vi "ReversedEngineering GetCompleteDependencyInfo.vi"(1 "path":path[](array[path]), 2 "SearchElements":T2[](array[typedef]), 4 "IgnoreClasses":path[](array[path]), 5 "error in (no error)":errorcluster, 6 "Only Create this class and its dependencis":bool, 7 "SyncOption":T1, 8 "Only analyse this class methods and attributes(False)":bool, 10 "CreateApplicationNode":bool) -> (15 "classInfos":T7[](array[typedef]), 16 "TypeDefs":T3[](array[typedef]), 17 "Cancelled":bool, 19 "error out":errorcluster)   [LabVIEW 2020]
doc: "Gets current diagram values"
uses:
  <resource>/Framework/Providers/Open_GDS/UML/ReversedEngineering/ReversedEngineering ClassInfoType.ctl
  <resource>/Framework/Providers/Open_GDS/ClassProviders/Common/CommonVIs/CommonVIs_VisibilityType.ctl
  <resource>/Framework/Providers/Open_GDS/ClassProviders/Common/CommonVIs/CommonVIs_AttributeInfoType.ctl
  <resource>/Framework/Providers/Open_GDS/ClassProviders/Common/CommonVIs/CommonVIs_AttributeDataType.ctl
  <resource>/Framework/Providers/Open_GDS/UML/ReversedEngineering/ReversedEngineering_ClassDependencyDetailsType.ctl
  <resource>/Framework/Providers/Open_GDS/ClassProviders/Common/ScriptingFunctions/SubVIs/Scripting_ViDependencyType.ctl
  <resource>/Framework/Providers/Open_GDS/ClassProviders/Common/CommonVIs/CommonVIs_TypeDefType.ctl
  <resource>/Framework/Providers/Open_GDS/UML/ReversedEngineering/ReversedEngineering RecursiveSearchElements.ctl
  <resource>/Framework/Providers/Open_GDS/UML/UMLEditor/UMLEditor_SyncOptions.ctl
  <resource>/Framework/Providers/Open_GDS/UML/UMLEditor/UMLEditor BusyDialogAction.ctl
  <resource>/Framework/Providers/Open_GDS/UML/UmlEditor_class/UmlEditor.lvclass
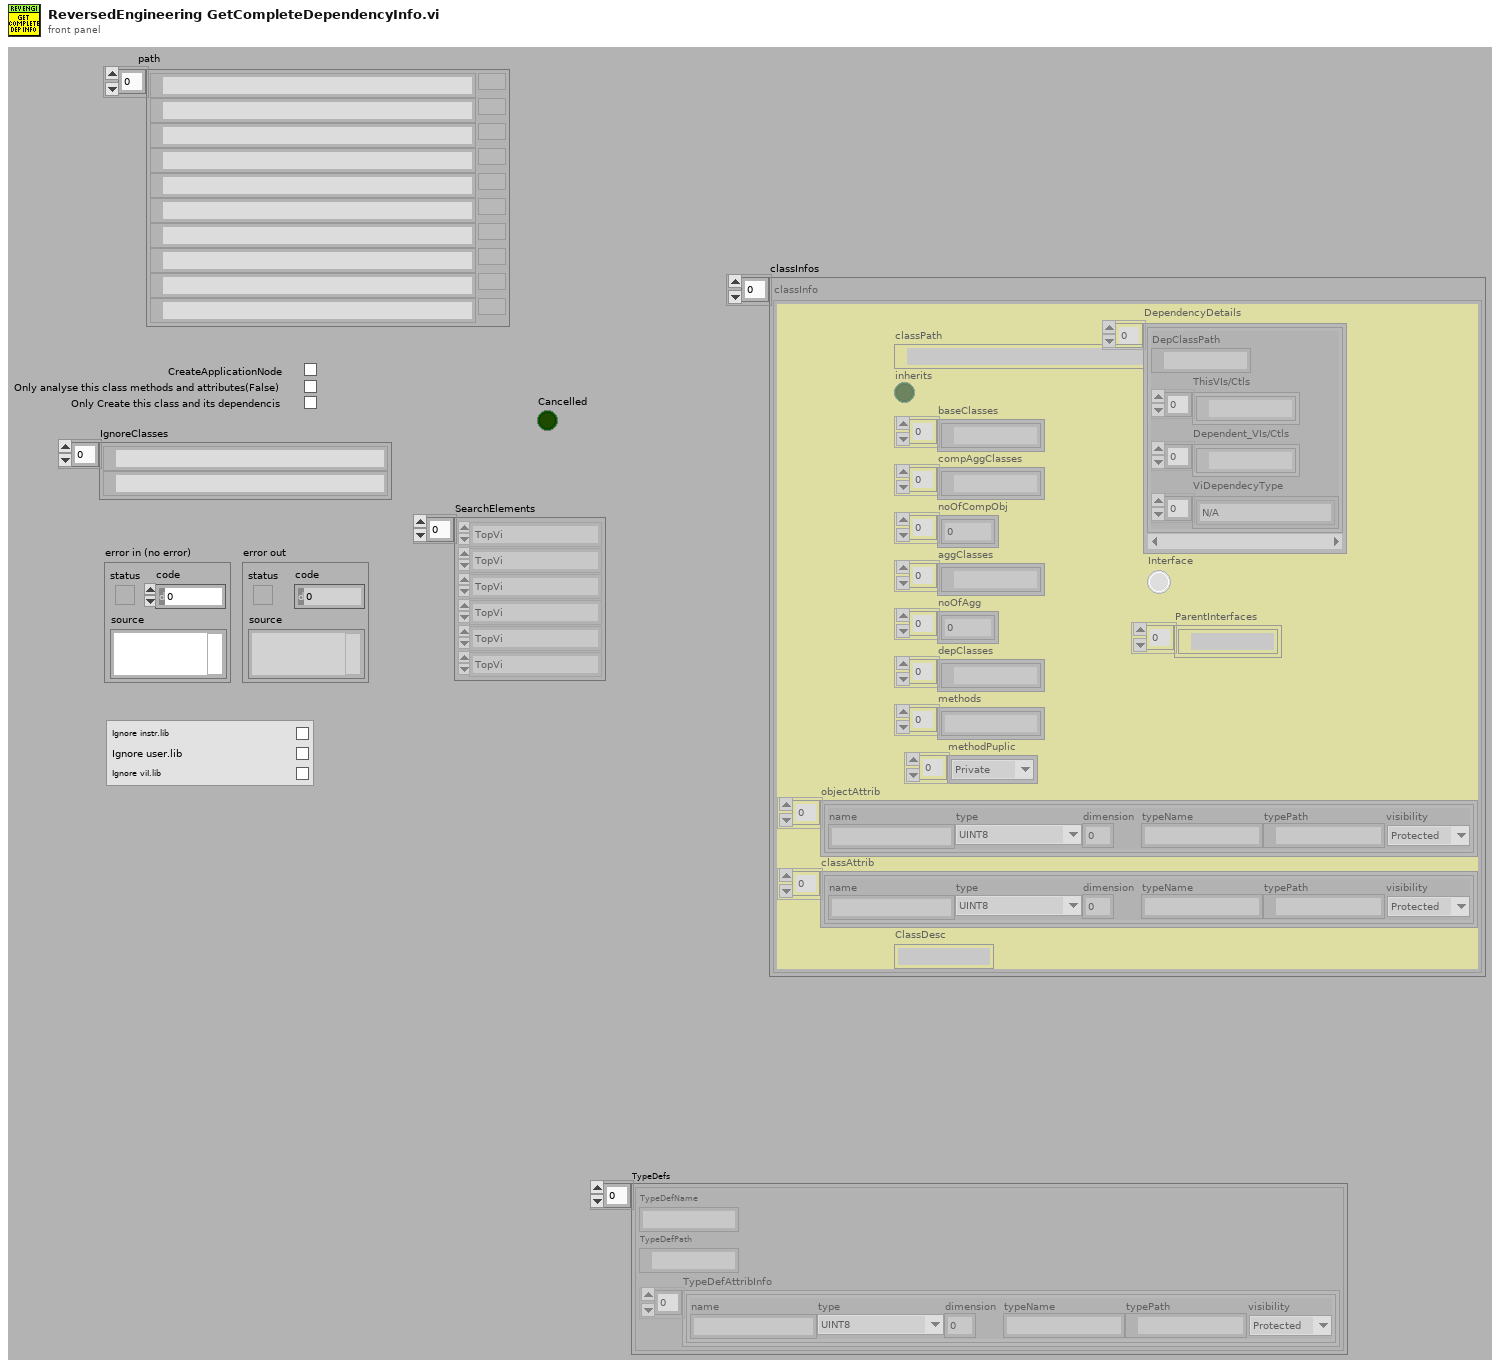
[diagram p1: front panel]
types:
  T1 = typedef "UMLEditor_SyncOptions.ctl" = cluster{"IgnoreInstrLib":bool, "IgnoreUserLib":bool, "IgnoreViLib":bool}
  T2 = typedef "ReversedEngineering RecursiveSearchElements.ctl" = enum16{"TopVi", "Class", "Dir", "Dir(rec.)"}
  T3 = typedef "CommonVIs_TypeDefType.ctl" = cluster{"TypeDefName":string, "TypeDefPath":path, "TypeDefAttribInfo":T4[]}
  T4 = typedef "CommonVIs_AttributeInfoType.ctl" = cluster{"name":string, "type":T5, "dimension":i32, "typeName":string, "typePath":path, "visibility":T6}
  T5 = typedef "CommonVIs_AttributeDataType.ctl" = enum16{"UINT8", "INT8", "UINT16", "INT16", "UINT32", "INT32", "UINT64", "INT64", "SGL", "DBL", "EXT", "CSG", "CDB", "CXT", "TimeStamp", "STRING", "PATH", "BOOL", "ENUM", "RefNum", "VIRefNum", "LabVIEW Class", "Cluster", "Variant", "TypeDef", "Waveform", "LabVIEW Object", "Other", "void", "Set", "Map"}
  T6 = typedef "CommonVIs_VisibilityType.ctl" = enum16{"Public", "Private", "Protected"}
  T7 = typedef "ReversedEngineering ClassInfoType.ctl" = cluster{"classPath":path, "inherits":bool, "baseClasses":path[], "compAggClasses":path[], "noOfCompObj":i32[], "aggClasses":path[], "noOfAgg":i32[], "depClasses":path[], "methods":string[], "methodPuplic":T6[], "objectAttrib":T4[], "classAttrib":T4[], "ClassDesc":string, "DependencyDetails":T8[], "Interface":bool, "ParentInterfaces":path[]}
  T8 = typedef "ReversedEngineering_ClassDependencyDetailsType.ctl" = cluster{"DepClassPath":path, "ThisVIs/Ctls":path[], "Dependent_VIs/Ctls":path[], "ViDependecyType":T9[]}
  T9 = typedef "Scripting_ViDependencyType.ctl" = enum16{"N/A", "Launches"}
  T10 = cluster{"dependencyClassPath":path[], "topVIPath":path, "classInfos":T7[], "calleesVIs":path[], "VIRef":refnum<vi>[], "TypeDefs":T3[], "TopVIPath":path, "SearchOnlyClasses":bool, "SearchDirs":path[], "SearchOnlyTopVIs":bool, "lvclasses":path[]}
  T11 = enum16{"Get Library Info", "Create Library Info", "Clear Library Info"}
  T12 = typedef "UMLEditor BusyDialogAction.ctl" = enum16{"Initialize", "Open(VIs)", "Open(i)", "Send_I-Value", "SendStatusMessage", "GetBusyDialogStatus", "Close", "Quit"}
  T13 = typedef "Librarian File Info Out.ctl" = cluster{"creation date":u32, "last mod date":u32, "type":string, "creator":string, "LV version":i32, "size":i32, "top level":bool}
  T14 = typedef "Scripting_VIClassDependency.ctl" = cluster{"VIPath":path, "Class":string, "ClassPath":path, "ViDependencyType":T9}
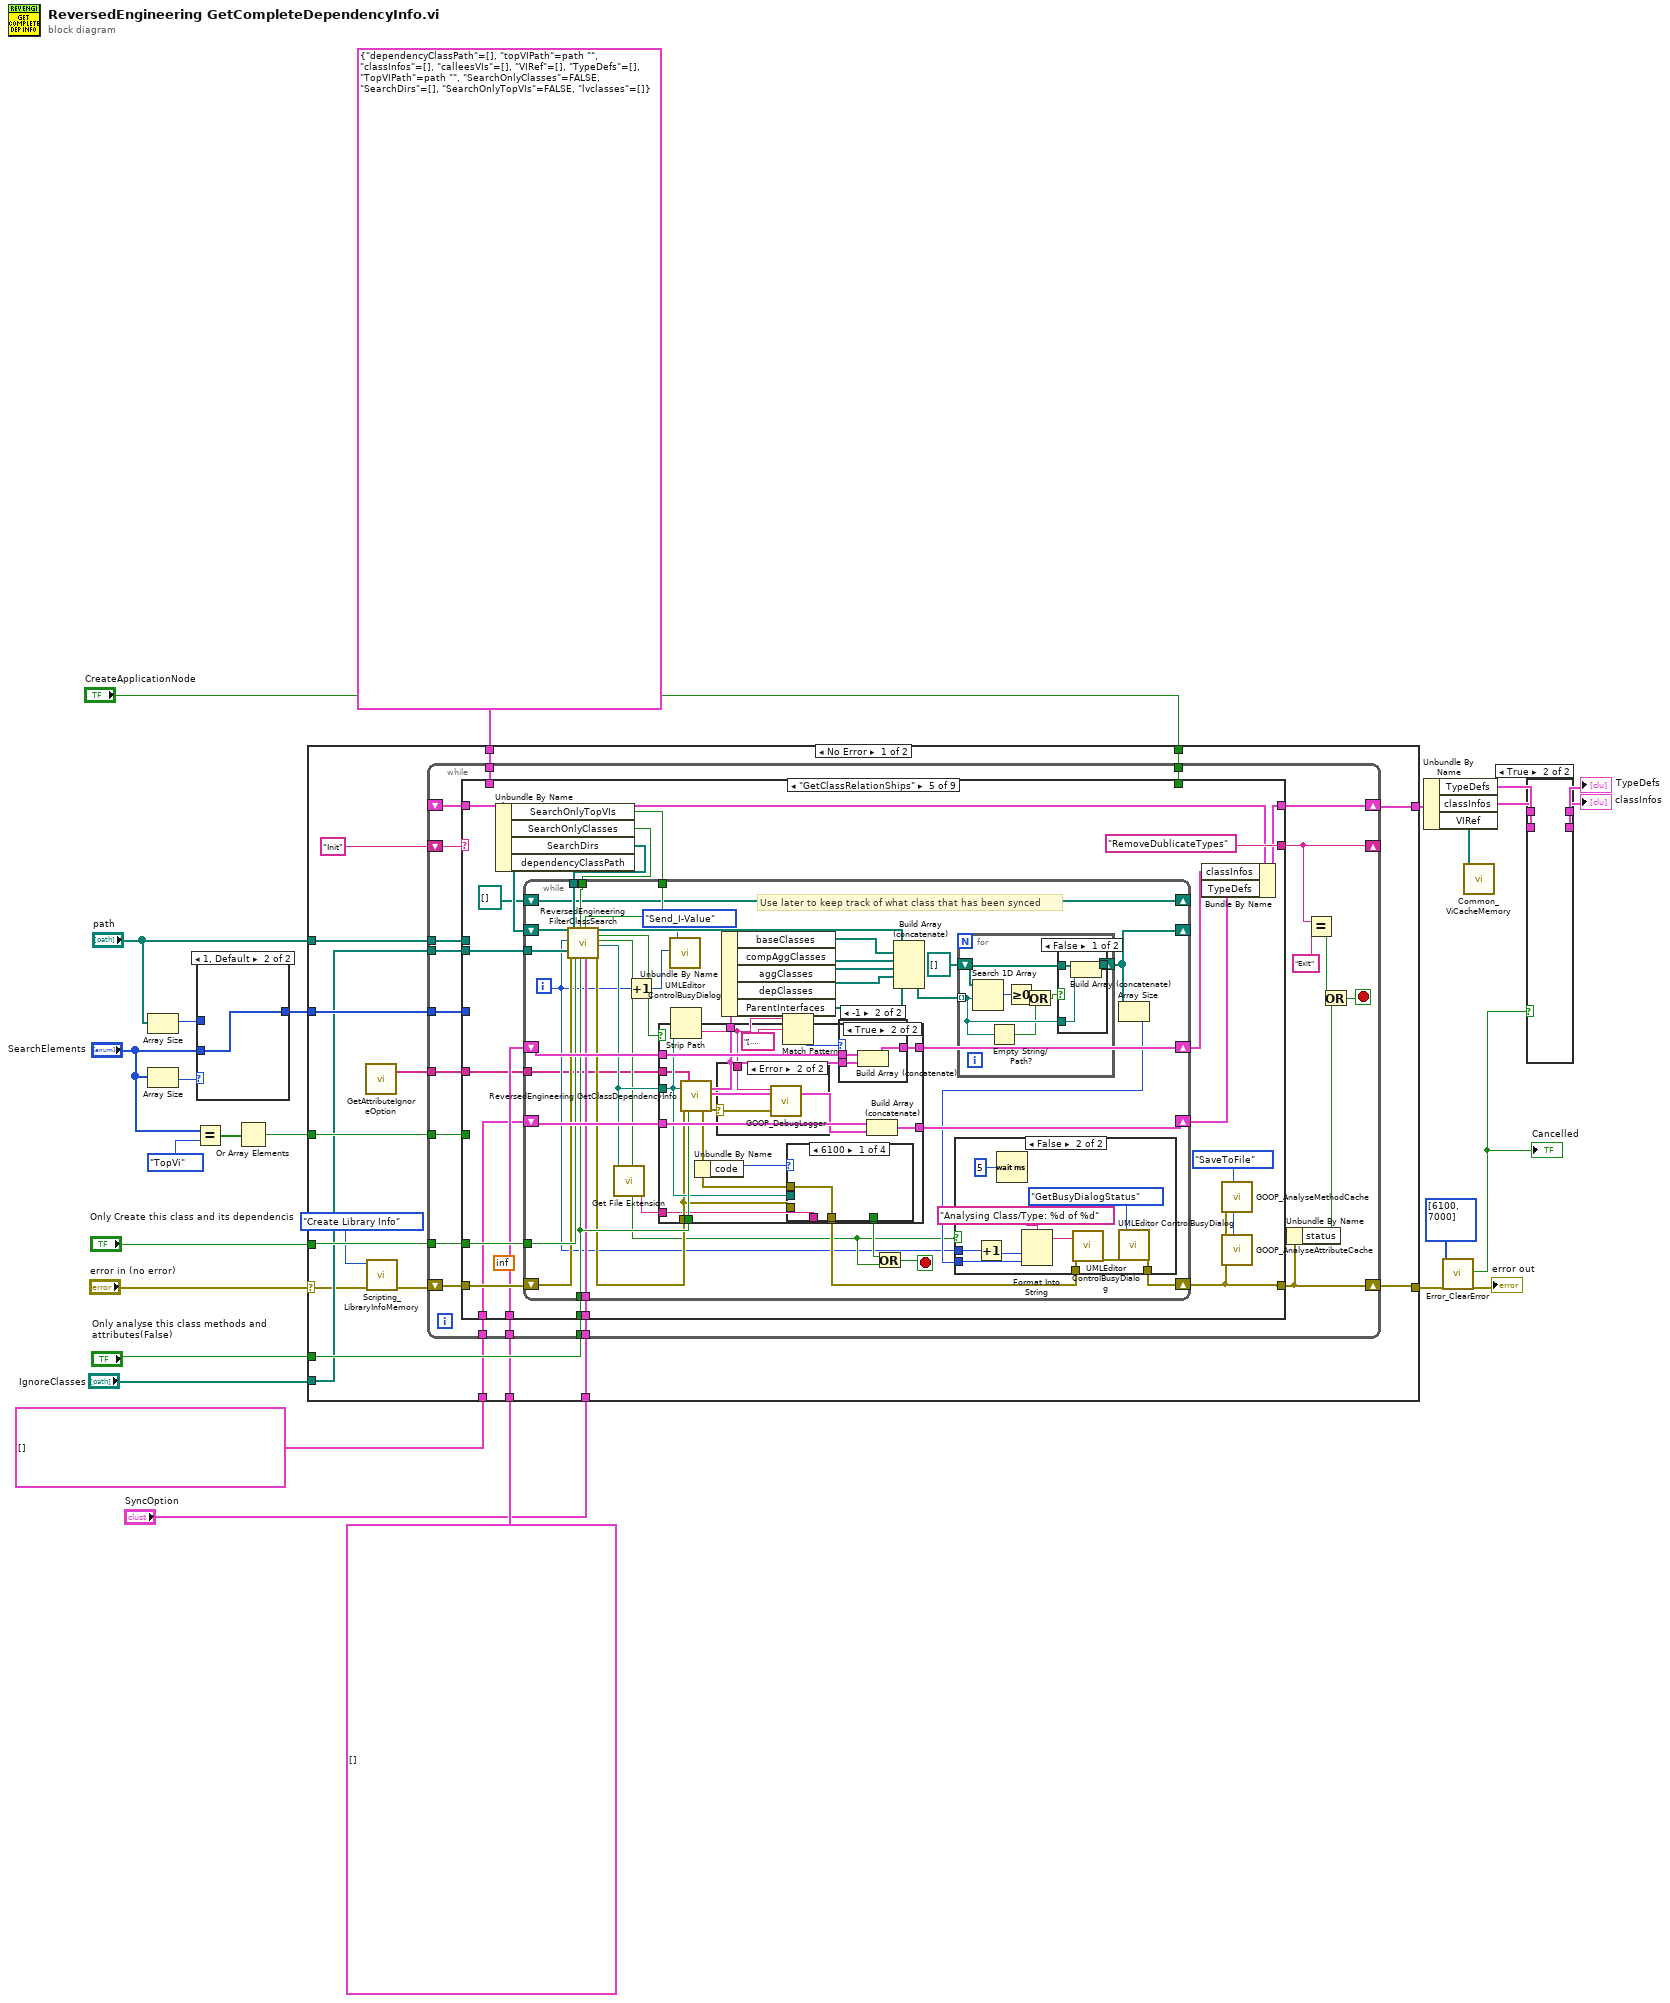
[diagram p0: block diagram]
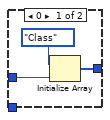
[diagram p3: hidden frame]
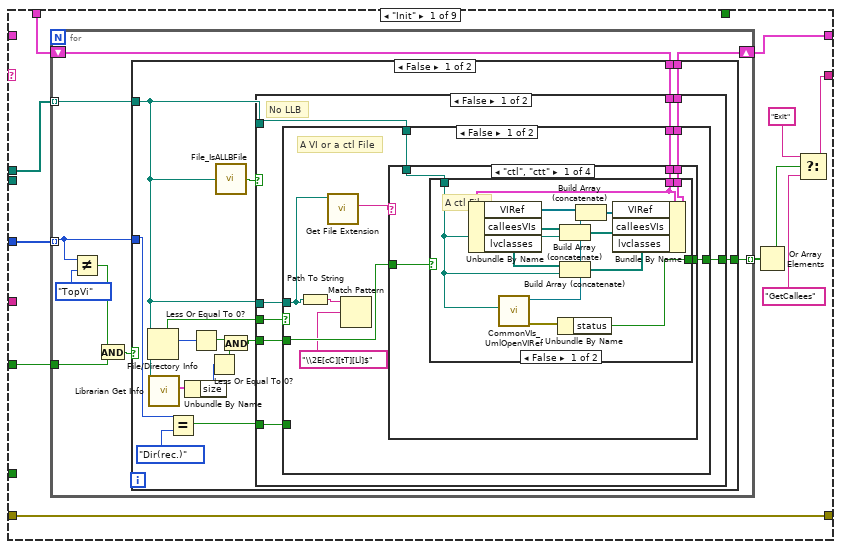
[diagram p4: hidden frame]
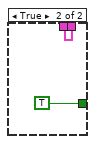
[diagram p5: hidden frame]
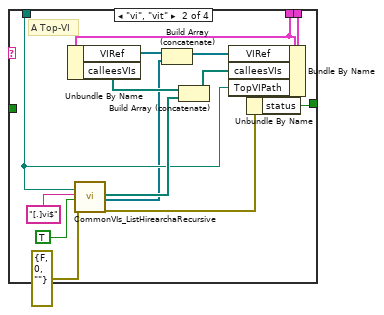
[diagram p6: hidden frame]
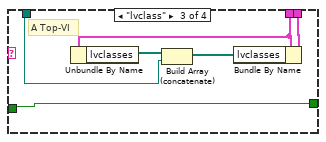
[diagram p7: hidden frame]
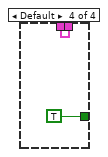
[diagram p8: hidden frame]
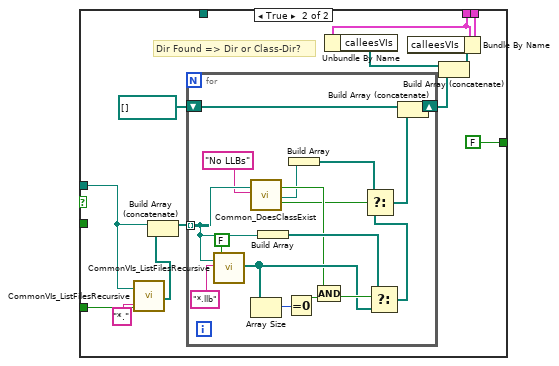
[diagram p9: hidden frame]
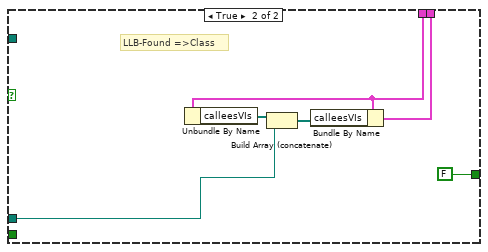
[diagram p10: hidden frame]
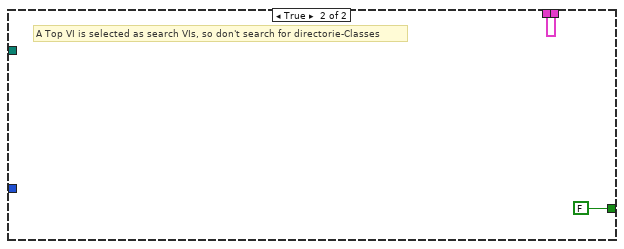
[diagram p11: hidden frame]
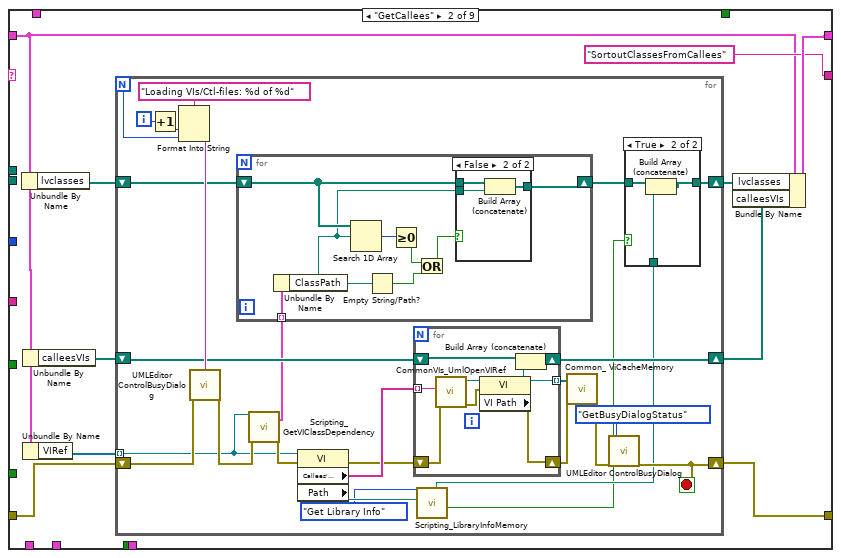
[diagram p12: hidden frame]
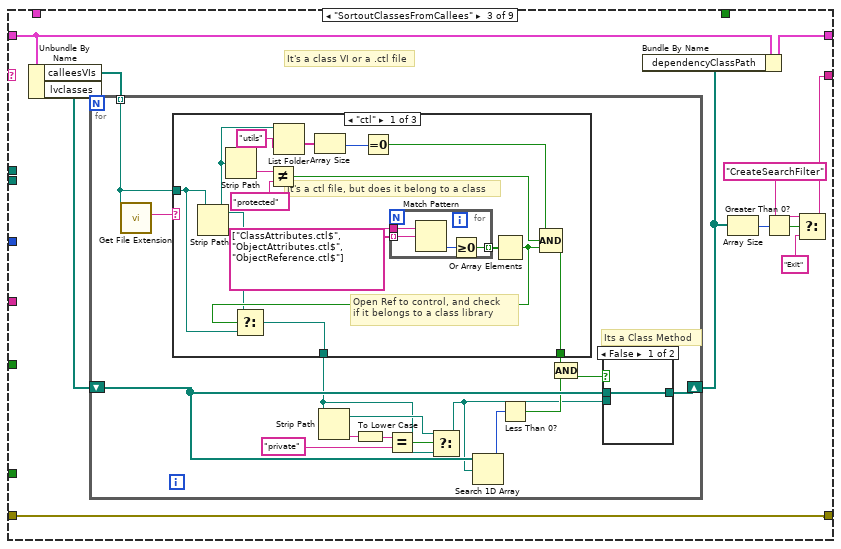
[diagram p15: hidden frame]
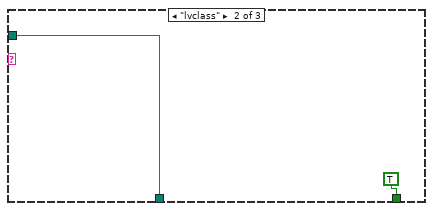
[diagram p16: hidden frame]
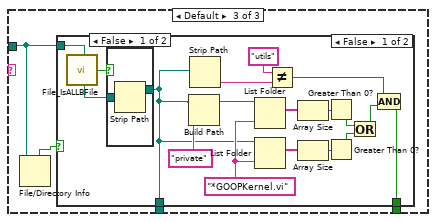
[diagram p17: hidden frame]
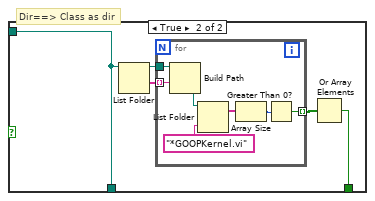
[diagram p19: hidden frame]
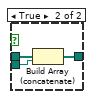
[diagram p20: hidden frame]
diagram:
  n1 = Array Size(array="path") -> (size(s)=w19:i32)
  n2 = Array Size(array="SearchElements") -> (size(s)=w21:i32)
  n3 = Equal?(x="SearchElements", y=ReversedEngineering_RecursiveSearchElements."TopVi" ("Enum")) -> (x = y?=w9:bool[])
  n4 = case shown="1, Default" w21 {
    tunnel: w19 -> [w29 _]
    tunnel: [w28 w31] -> w18
    tunnel: "SearchElements" -> [_ w31]
    frame 0 {
      n5 = Initialize Array(ReversedEngineering_RecursiveSearchElements."Class" ("Enum"), w29) -> (w28:T2[])
    }
    frame 1, Default {
    }
  }
  n6 = Or Array Elements(Boolean array=w9) -> (logical OR=w7:bool)
  n7 = case shown="No Error" "error in (no error)" {
    selector: "error in (no error)" -> [w35 w642]
    tunnel: [w48 w642] -> w17
    tunnel: "path" -> [w47 _]
    tunnel: [w46 _] -> w26
    tunnel: "Only Create this class and its dependencis" -> [w45 _]
    tunnel: "Only analyse this class methods and attributes(False)" -> [w42 _]
    tunnel: "CreateApplicationNode" -> [w44 _]
    tunnel: w18 -> [w43 _]
    tunnel: w7 -> [w41 _]
    tunnel: T10 {"dependencyClassPath"=[], "topVIPath"=path "", "classInfos"=[], "calleesVIs"=[], "VIRef"=[], "TypeDefs"=[], "TopVIPath"=path "", "SearchOnlyClasses"=FALSE, "SearchDirs"=[], "SearchOnlyTopVIs"=FALSE, "lvclasses"=[]} ("Cluster") -> [w40 _]
    tunnel: T7[] [] -> [w39 _]
    tunnel: T3[] [] -> [w38 _]
    tunnel: "IgnoreClasses" -> [w37 _]
    tunnel: "SyncOption" -> [w36 _]
    frame No Error {
      n8 = call <resource>:"GetAttributeIgnoreOption.vi"() -> ("Attr"=w32:string[])  [unwired: 1 in, 18 out]
      n9 = call <resource>:"Scripting_LibraryInfoMemory.vi"("error in (no error)"=w35, "Action"=T11."Create Library Info") -> ("error out"=w34:errorcluster)  [unwired: 5 in, 4 out]
      n10 = while {
        shift-right: [w68] -> _
        shift-left: "Init" -> [w71]
        shift-right: [w69] -> w48
        shift-left: w34 -> [w70]
        shift-right: [w62] -> w46
        shift-left: _ -> [w63]
        tunnel: w47 -> [w61]
        tunnel: w45 -> [w60]
        tunnel: w44 -> [w59]
        tunnel: w43 -> [w58]
        tunnel: w42 -> [w57]
        tunnel: w41 -> [w56]
        tunnel: w40 -> [w55]
        tunnel: w39 -> [w54]
        tunnel: w38 -> [w53]
        tunnel: w37 -> [w52]
        tunnel: w36 -> [w51]
        tunnel: w32 -> [w50]
        stop <- w64 stop-if-true
        n11 = case shown="\"GetClassRelationShips\"" w71 {
          tunnel: w70 -> [w82 w207 w271 w353 w419 w528 w559 w631 w639]
          tunnel: [w82 w208 w271 w350 w405 w528 w559 w631 w639] -> w69
          tunnel: [w81 "SortoutClassesFromCallees" ("y") w266 "GetClassRelationShips" ("y") "RemoveDublicateTypes" ("y") "RemoveClassDependenciesDueToInheritance" ("y") w555 "Exit" ("y") "Exit" ("y")] -> w68
          tunnel: w63 -> [_ w204 w270 w365 w420 w531 w561 w630 w641]
          tunnel: [w75 w210 w272 w364 w421 w529 w560 w629 w641] -> w62
          tunnel: w61 -> [w80 _ _ w360 _ _ _ _ _]
          tunnel: w60 -> [_ _ _ _ w416 _ _ _ _]
          tunnel: w59 -> [_ _ _ _ _ _ w553 _ _]
          tunnel: w58 -> [w74 _ _ w355 _ _ _ _ _]
          tunnel: w57 -> [_ _ _ _ w414 _ _ _ _]
          tunnel: w56 -> [w73 _ _ _ _ _ _ _ _]
          tunnel: w55 -> [w72 _ _ _ _ _ _ _ _]
          tunnel: w54 -> [_ _ _ _ w410 _ _ _ _]
          tunnel: w53 -> [_ _ _ _ w409 _ _ _ _]
          tunnel: w52 -> [_ _ _ _ w407 _ _ _ _]
          tunnel: w51 -> [_ _ _ _ w406 _ _ _ _]
          tunnel: w50 -> [_ _ _ _ w403 _ _ _ _]
          frame "Init" {
            n12 = for {
              tunnel: w80 -> [w88] mode=indexing
              shift-right: [w90] -> w75
              shift-left: w72 -> [w91]
              tunnel: [w89] -> w79 mode=indexing
              tunnel: w74 -> [w87] mode=indexing
              tunnel: w73 -> [w83]
              n13 = Not Equal?(x=w87, y=ReversedEngineering_RecursiveSearchElements."TopVi") -> (x != y?=w85:bool)
              n14 = And(x=w85, y=w83) -> (x .and. y?=w84:bool)
              n15 = case shown="False" w84 {
                tunnel: w91 -> [w106 w200]
                tunnel: [w105 w200] -> w90
                tunnel: [w104 FALSE ("status")] -> w89
                tunnel: w88 -> [w96 _]
                tunnel: w87 -> [w99 _]
                frame False {
                  n16 = File/Directory Info(path=w96) -> (directory=w102:bool, size=w98:i64)  [unwired: 1 in, 5 out]
                  n17 = call <vilib>:"Librarian Get Info.vi"("path"=w96) -> ("file information"=w95:T13)  [unwired: 1 in, 9 out]
                  n18 = Equal?(x=w99, y=ReversedEngineering_RecursiveSearchElements."Dir(rec.)") -> (x = y?=w100:bool)
                  n19 = Unbundle By Name(w95) -> ("size"=w94:i32)
                  n20 = Less Or Equal To 0?(x=w98) -> (x <= 0?=w97:bool)
                  n21 = Less Or Equal To 0?(x=w94) -> (x <= 0?=w93:bool)
                  n22 = call <resource>:"File_IsALLBFile.vi"("path"=w96) -> ("path to VI library?"=w103:bool)
                  n23 = And(x=w97, y=w93) -> (x .and. y?=w92:bool)
                  n24 = case shown="False" w103 {
                    tunnel: w92 -> [w114 _]
                    tunnel: w96 -> [w113 _]
                    tunnel: w106 -> [w112 w196]
                    tunnel: [w111 w197] -> w105
                    tunnel: [w110 FALSE ("status")] -> w104
                    tunnel: w96 -> [w108 w195]
                    tunnel: w102 -> [w109 _]
                    tunnel: w100 -> [w107 _]
                    frame False {
                      # "No LLB"
                      n25 = case shown="False" w109 {
                        tunnel: w114 -> [w123 _]
                        tunnel: w113 -> [w122 _]
                        tunnel: w112 -> [w121 w174]
                        tunnel: [w120 w173] -> w111
                        tunnel: [w119 FALSE] -> w110
                        tunnel: w108 -> [w116 w169]
                        tunnel: w107 -> [_ w170]
                        frame False {
                          # "A VI or a ctl File"
                          n26 = Path To String(path=w116) -> (string=w118:string)
                          n27 = call <vilib>:"Get File Extension.vi"("file"=w116) -> ("lowercase file extension"=w115:string)  [unwired: 1 in, 9 out]
                          n28 = Match Pattern(string=w118, regular expression="\\2E[cC][tT][Ll]$") -> ()  [unwired: 5 out]
                          n29 = case shown="\"ctl\", \"ctt\"" w115 {
                            tunnel: w123 -> [w128 _ w157 _]
                            tunnel: w122 -> [w127 w145 w158 _]
                            tunnel: w121 -> [w126 w154 w160 w164]
                            tunnel: [w125 w153 w159 w164] -> w120
                            tunnel: [w124 w150 w157 TRUE ("status")] -> w119
                            frame "ctl", "ctt" {
                              n30 = case shown="False" w128 {
                                tunnel: w127 -> [w129 _]
                                tunnel: w126 -> [w136 w142]
                                tunnel: [w138 w142] -> w125
                                tunnel: [w134 TRUE] -> w124
                                frame False {
                                # "A ctl File"
                                n31 = Unbundle By Name(w136) -> ("VIRef"=w139:refnum<vi>[], "calleesVIs"=w133:path[], "lvclasses"=w131:path[])
                                n32 = call <resource>:"CommonVIs_UmlOpenVIRef.vi"("ViPath/ViName"=w129) -> ("error out"=w135:errorcluster, "vi reference"=w137:refnum<vi>)  [unwired: 3 in, 6 out]
                                n33 = Unbundle By Name(w135) -> ("status"=w134:bool)
                                n34 = Build Array (concatenate)(w133, w129) -> (w132:path[])
                                n35 = Build Array (concatenate)(w131, w129) -> (w130:path[])
                                n36 = Build Array (concatenate)(w139, w137) -> (w140:refnum<vi>[])
                                n37 = Bundle By Name(cluster=w136, "VIRef"=w140, "calleesVIs"=w132, "lvclasses"=w130) -> (w138:T10)
                                }
                                frame True {
                                }
                              }
                            }
                            frame "vi", "vit" {
                              # "A Top-VI"
                              n38 = Unbundle By Name(w154) -> ("VIRef"=w155:refnum<vi>[], "calleesVIs"=w152:path[])
                              n39 = call <resource>:"CommonVIs_ListHirearchaRecursive.vi"("FilePath"=w145, "FileSearchPattern"="[.]vi$", "IgnoreClassMemberVIs(False)"=TRUE ("IgnoreClassMemberVIs(Flase)"), "error in (no error)"=errorcluster {"status"=FALSE, "code"=0, "source"=""}) -> ("Files"=w147:path[], "VIRefs"=w144:refnum<vi>[], "error out"=w146:errorcluster)  [unwired: 13 out]
                              n40 = Build Array (concatenate)(w155, w144) -> (w156:refnum<vi>[])
                              n41 = Build Array (concatenate)(w152, w147) -> (w151:path[])
                              n42 = Bundle By Name(cluster=w154, "VIRef"=w156, "calleesVIs"=w151, "TopVIPath"=w145) -> (w153:T10)
                              n43 = Unbundle By Name(w146) -> ("status"=w150:bool)
                            }
                            frame "lvclass" {
                              # "A Top-VI"
                              n44 = Unbundle By Name(w160) -> ("lvclasses"=w161:path[])
                              n45 = Build Array (concatenate)(w161, w158) -> (w162:path[])
                              n46 = Bundle By Name(cluster=w160, "lvclasses"=w162) -> (w159:T10)
                            }
                            frame Default {
                            }
                          }
                        }
                        frame True {
                          # "Dir Found => Dir or Class-Dir?"
                          n47 = call <resource>:"CommonVIs_ListFilesRecursive.vi"("directory path"=w169, "FileSearchPattern"="*." ("pattern"), "RecusiveSearch(True)"=w170) -> ("Directories"=w168:path[])  [unwired: 3 in, 13 out]
                          n48 = Build Array (concatenate)(w169, w168) -> (w167:path[])
                          n49 = for {
                            tunnel: w167 -> [w184] mode=indexing
                            shift-right: [w189] -> w165
                            shift-left: path[] [] ("calleesVIs") -> [w188]
                            n50 = call <resource>:"CommonVIs_ListFilesRecursive.vi"("directory path"=w184, "FileSearchPattern"="*.llb" ("pattern"), "RecusiveSearch(True)"=FALSE ("RecusiveSerach(True)")) -> ("Files"=w186:path[])  [unwired: 3 in, 13 out]
                            n51 = call <resource>:"Common_DoesClassExist.vi"("ClassPath"=w184, "ClassName"="No LLBs") -> ("ClassExists"=w183:bool, "llb/LvCLass-Path"=w181:path, "LvClassExists"=w180:bool)  [unwired: 15 out]
                            n52 = Array Size(array=w186) -> (size(s)=w193:i32)
                            n53 = Build Array(w184) -> (w185:path[])
                            n54 = Equal To 0?(x=w193) -> (x = 0?=w192:bool)
                            n55 = Build Array(w181) -> (w179:path[])
                            n56 = Compound Arithmetic op=AND(w183, w192) -> (w187:bool)
                            n57 = Select(t=w185, s=w187, f=w186) -> (s? t:f=w177:path[])
                            n58 = Select(t=w179, s=w180, f=w177) -> (s? t:f=w178:path[])
                            n59 = Build Array (concatenate)(w188, w178) -> (w189:path[])
                          }
                          n60 = Unbundle By Name(w174) -> ("calleesVIs"=w176:path[])
                          n61 = Build Array (concatenate)(w176, w165) -> (w175:path[])
                          n62 = Bundle By Name(cluster=w174, "calleesVIs"=w175) -> (w173:T10)
                        }
                      }
                    }
                    frame True {
                      # "LLB-Found =>Class"
                      n63 = Unbundle By Name(w196) -> ("calleesVIs"=w199:path[])
                      n64 = Build Array (concatenate)(w199, w195) -> (w198:path[])
                      n65 = Bundle By Name(cluster=w196, "calleesVIs"=w198) -> (w197:T10)
                    }
                  }
                }
                frame True {
                  # "A Top VI is selected as search VIs, so don't search for directorie-Classes"
                }
              }
            }
            n66 = Or Array Elements(Boolean array=w79) -> (logical OR=w78:bool)
            n67 = Select(t="Exit", s=w78, f="GetCallees") -> (s? t:f=w81:string)
          }
          frame "GetCallees" {
            n68 = Unbundle By Name(w204) -> ("lvclasses"=w203:path[])
            n69 = Unbundle By Name(w204) -> ("calleesVIs"=w205:path[])
            n70 = Unbundle By Name(w204) -> ("VIRef"=w211:refnum<vi>[])
            n71 = for {
              N -> [w232]
              tunnel: w211 -> [w216] mode=indexing
              shift-right: [w236] -> w206
              shift-left: w205 -> [w226]
              shift-right: [w219] -> w208
              shift-left: w207 -> [w218]
              shift-right: [w220] -> w202
              shift-left: w203 -> [w223]
              i -> [w234]
              stop <- w219 stop-if-true
              n72 = Increment(x=w234) -> (x+1=w233:i32)
              n73 = Format Into String(format string="Loading VIs/Ctl-files: %d of %d", w233, w232) -> (resulting string=w231:string)  [unwired: 2 in, 1 out]
              n74 = call <resource>:"UMLEditor ControlBusyDialog.vi"("Title/StatusText"=w231, "error in (no error)"=w218) -> ("error out"=w217:errorcluster)  [unwired: 2 in, 15 out]
              n75 = call <resource>:"Scripting_GetVIClassDependency.vi"("ViRef"=w216, "error in (no error)"=w217) -> ("DepVIs"=w224:T14[], "error out"=w225:errorcluster)  [unwired: 16 out]
              n76 = for {
                tunnel: w224 -> [w248] mode=indexing
                shift-right: [w249] -> w221
                shift-left: w223 -> [w247]
                n77 = Unbundle By Name(w248) -> ("ClassPath"=w245:path)
                n78 = Search 1D Array(1D array=w247, element=w245) -> (index of element=w246:i32)  [unwired: 1 out]
                n79 = Empty String/Path?(string/path=w245) -> (empty?=w243:bool)
                n80 = Greater Or Equal To 0?(x=w246) -> (x >= 0?=w244:bool)
                n81 = Or(x=w244, y=w243) -> (x .or. y?=w242:bool)
                n82 = case shown="False" w242 {
                  tunnel: w247 -> [w250 w253]
                  tunnel: [w250 w252] -> w249
                  tunnel: w245 -> [_ w251]
                  frame True {
                  }
                  frame False {
                    n83 = Build Array (concatenate)(w253, w251) -> (w252:path[])
                  }
                }
              }
              n84 = property class="VI"(reference=w216, error in=w225) -> (error out=w222:errorcluster, "Callees' Names"=w237:string[], "Path"=w215:path)  [unwired: 1 out]
              n85 = for {
                tunnel: w237 -> [w256] mode=indexing
                shift-right: [w260] -> w236
                shift-left: w226 -> [w262]
                shift-right: [w255] -> w228
                shift-left: w222 -> [w261]
                tunnel: [w254] -> w229 mode=indexing
                n86 = call <resource>:"CommonVIs_UmlOpenVIRef.vi"("error in"=w261, "ViPath/ViName"=w256) -> ("error out"=w258:errorcluster, "vi reference"=w259:refnum<vi>)  [unwired: 2 in, 6 out]
                n87 = property class="VI"(reference=w259, error in=w258) -> (reference out=w254:refnum<vi>, error out=w255:errorcluster, "VI Path"=w257:path)
                n88 = Build Array (concatenate)(w262, w257) -> (w260:path[])
              }
              n89 = call <resource>:"Scripting_LibraryInfoMemory.vi"("ViPath"=w215, "Action"=T11."Get Library Info") -> ("Found"=w213:bool, "LibaryPath"=w214:path)  [unwired: 5 in, 3 out]
              n90 = call <resource>:"Common_ ViCacheMemory.vi"("ViRef-Array"=w229, "error in (no error)"=w228) -> ("error out"=w227:errorcluster)  [unwired: 2 in, 15 out]
              n91 = call <resource>:"UMLEditor ControlBusyDialog.vi"("error in (no error)"=w227, "Action(SendStatusMessage)"=UMLEditor_BusyDialogAction."GetBusyDialogStatus") -> ("error out"=w219:errorcluster)  [unwired: 2 in, 15 out]
              n92 = case shown="True" w213 {
                tunnel: w221 -> [w238 w241]
                tunnel: w214 -> [_ w240]
                tunnel: [w238 w239] -> w220
                frame False {
                }
                frame True {
                  n93 = Build Array (concatenate)(w241, w240) -> (w239:path[])
                }
              }
            }
            n94 = Bundle By Name(cluster=w204, "lvclasses"=w202, "calleesVIs"=w206) -> (w210:T10)
          }
          frame "SortoutClassesFromCallees" {
            # "It's a class VI or a .ctl file"
            n95 = Unbundle By Name(w270) -> ("calleesVIs"=w273:path[], "lvclasses"=w263:path[])
            n96 = for {
              tunnel: w273 -> [w275] mode=indexing
              shift-right: [w286] -> w269
              shift-left: w263 -> [w287]
              # "Its a Class Method"
              n97 = call <vilib>:"Get File Extension.vi"("file"=w275) -> ("lowercase file extension"=w274:string)  [unwired: 1 in, 9 out]
              n98 = case shown="\"ctl\"" w274 {
                tunnel: [w295 TRUE w313] -> w283
                tunnel: [w303 w309 w312] -> w276
                tunnel: w275 -> [w299 w309 w310]
                frame "ctl" {
                  # "Open Ref to control, and check\nif it belongs to a class library"
                  # "It's a ctl file, but does it belong to a class"
                  n99 = Strip Path(path=w299) -> (stripped path=w293:path, name=w302:string)
                  n100 = Strip Path(path=w293) -> (name=w298:string)  [unwired: 1 out]
                  n101 = Not Equal?(x=w298, y="protected") -> (x != y?=w294:bool)
                  n102 = List Folder(path=w293, pattern="utils" ("y")) -> (folder names=w292:string[])  [unwired: 1 in, 4 out]
                  n103 = Array Size(array=w292) -> (size(s)=w290:i32)
                  n104 = Equal To 0?(x=w290) -> (x = 0?=w289:bool)
                  n105 = for {
                    tunnel: w302 -> [w307]
                    tunnel: string[] ["ClassAttributes.ctl$", "ObjectAttributes.ctl$", "ObjectReference.ctl$"] -> [w306] mode=indexing
                    tunnel: [w304] -> w300 mode=indexing
                    n106 = Match Pattern(string=w307, regular expression=w306) -> (offset past match=w305:i32)  [unwired: 4 out]
                    n107 = Greater Or Equal To 0?(x=w305) -> (x >= 0?=w304:bool)
                  }
                  n108 = Or Array Elements(Boolean array=w300) -> (logical OR=w296:bool)
                  n109 = Select(t=w293, s=w296, f=w299) -> (s? t:f=w303:path)
                  n110 = Compound Arithmetic op=AND(w289, w294, w296) -> (w295:bool)
                }
                frame "lvclass" {
                }
                frame Default {
                  n111 = File/Directory Info(path=w310) -> (directory=w311:bool)  [unwired: 1 in, 6 out]
                  n112 = case shown="False" w311 {
                    tunnel: [w314 w334] -> w313
                    tunnel: [w319 w338] -> w312
                    tunnel: w310 -> [w326 w338]
                    frame False {
                      w321 = "*GOOPKernel.vi" ("pattern")
                      n113 = call <resource>:"File_IsALLBFile.vi"("path"=w326) -> ("path to VI library?"=w330:bool)
                      n114 = case shown="False" w330 {
                        tunnel: [w332 w333] -> w319
                        tunnel: w326 -> [w331 w333]
                        frame False {
                          n115 = Strip Path(path=w331) -> (stripped path=w332:path)  [unwired: 1 out]
                        }
                        frame True {
                        }
                      }
                      n116 = Build Path(base path=w319, name or relative path="private") -> (appended path=w320:path)
                      n117 = Strip Path(path=w319) -> (name=w318:string)  [unwired: 1 out]
                      n118 = List Folder(path=w320, pattern=w321) -> (filenames=w325:string[])  [unwired: 1 in, 4 out]
                      n119 = List Folder(path=w319, pattern=w321) -> (filenames=w328:string[])  [unwired: 1 in, 4 out]
                      n120 = Not Equal?(x="utils" ("name or relative path"), y=w318) -> (x != y?=w316:bool)
                      n121 = Array Size(array=w325) -> (size(s)=w324:i32)
                      n122 = Array Size(array=w328) -> (size(s)=w329:i32)
                      n123 = Greater Than 0?(x=w324) -> (x > 0?=w323:bool)
                      n124 = Greater Than 0?(x=w329) -> (x > 0?=w327:bool)
                      n125 = Or(x=w323, y=w327) -> (x .or. y?=w315:bool)
                      n126 = Compound Arithmetic op=AND(w316, w315) -> (w314:bool)
                    }
                    frame True {
                      # "Dir==> Class as dir"
                      n127 = List Folder(path=w338) -> (path out=w337:path, folder names=w335:string[])  [unwired: 1 in, 4 out]
                      n128 = for {
                        tunnel: w337 -> [w342]
                        tunnel: [w340] -> w336 mode=indexing
                        tunnel: w335 -> [w339] mode=indexing
                        n129 = Build Path(base path=w342, name or relative path=w339) -> (appended path=w341:path)
                        n130 = List Folder(path=w341, pattern="*GOOPKernel.vi") -> (filenames=w344:string[])  [unwired: 1 in, 4 out]
                        n131 = Array Size(array=w344) -> (size(s)=w345:i32)
                        n132 = Greater Than 0?(x=w345) -> (x > 0?=w340:bool)
                      }
                      n133 = Or Array Elements(Boolean array=w336) -> (logical OR=w334:bool)
                    }
                  }
                }
              }
              n134 = Strip Path(path=w276) -> (stripped path=w278:path, name=w282:string)
              n135 = To Lower Case(string=w282) -> (all lower case string=w281:string)
              n136 = Equal?(x=w281, y="private" ("name or relative path")) -> (x = y?=w279:bool)
              n137 = Select(t=w278, s=w279, f=w276) -> (s? t:f=w277:path)
              n138 = Search 1D Array(1D array=w287, element=w277) -> (index of element=w288:i32)  [unwired: 1 out]
              n139 = Less Than 0?(x=w288) -> (x < 0?=w284:bool)
              n140 = Compound Arithmetic op=AND(w283, w284) -> (w285:bool)
              n141 = case shown="False" w285 {
                tunnel: w287 -> [w346 w349]
                tunnel: [w346 w348] -> w286
                tunnel: w277 -> [_ w347]
                frame False {
                }
                frame True {
                  n142 = Build Array (concatenate)(w349, w347) -> (w348:path[])
                }
              }
            }
            n143 = Bundle By Name(cluster=w270, "dependencyClassPath"=w269) -> (w272:T10)
            n144 = Array Size(array=w269) -> (size(s)=w268:i32)
            n145 = Greater Than 0?(x=w268) -> (x > 0?=w267:bool)
            n146 = Select(t="CreateSearchFilter" ("y"), s=w267, f="Exit" ("y")) -> (s? t:f=w266:string)
          }
          frame "CreateSearchFilter" {
            n147 = for {
              tunnel: w355 -> [w370] mode=indexing
              tunnel: w360 -> [w369] mode=indexing
              shift-right: [w371] -> w358
              shift-left: path[] [] -> [w372]
              n148 = case shown="\"Class\"" w370 {
                tunnel: w372 -> [w373 w381 w396 w402]
                tunnel: [w373 w380 w395 w401] -> w371
                tunnel: w369 -> [_ w377 w392 w397]
                frame Default {
                }
                frame "Dir" {
                  n149 = call <resource>:"CommonVIs_ListFilesRecursive.vi"("directory path"=w377, "FileSearchPattern"="*." ("pattern"), "RecusiveSearch(True)"=FALSE ("RecusiveSerach(True)")) -> ("Directories"=w376:path[])  [unwired: 3 in, 13 out]
                  n150 = for {
                    tunnel: w376 -> [w383] mode=indexing
                    shift-right: [w385] -> w374
                    shift-left: path[] [] ("f") -> [w384]
                    n151 = call <resource>:"Common_DoesClassExist.vi"("ClassPath"=w383, "ClassName"="No LLBs") -> ("ClassExists"=w382:bool)  [unwired: 17 out]
                    n152 = case shown="False" w382 {
                      tunnel: [w387 w390] -> w385
                      tunnel: w384 -> [w387 w389]
                      tunnel: w383 -> [_ w388]
                      frame False {
                      }
                      frame True {
                        n153 = Build Array (concatenate)(w389, w388) -> (w390:path[])
                      }
                    }
                  }
                  n154 = Build Array (concatenate)(w381, w377, w374) -> (w380:path[])
                }
                frame "Class" {
                  n155 = File/Directory Info(path=w392) -> (directory=w393:bool)  [unwired: 1 in, 6 out]
                  n156 = Strip Path(path=w392) -> (stripped path=w391:path)  [unwired: 1 out]
                  n157 = Select(t=w392, s=w393, f=w391) -> (s? t:f=w394:path)
                  n158 = Build Array (concatenate)(w396, w394) -> (w395:path[])
                }
                frame "Dir(rec.)" {
                  n159 = call <resource>:"CommonVIs_ListFilesRecursive.vi"("directory path"=w397, "FileSearchPattern"="*.", "SearchInLLBs(True)"=FALSE) -> ("Directories"=w400:path[])  [unwired: 3 in, 13 out]
                  n160 = Build Array (concatenate)(w402, w397, w400) -> (w401:path[])
                }
              }
            }
            n161 = Equal?(x=w355, y=ReversedEngineering_RecursiveSearchElements."TopVi" ("Enum")) -> (x = y?=w357:bool[])
            n162 = Equal?(x=w355, y=ReversedEngineering_RecursiveSearchElements."Class" ("Enum")) -> (x = y?=w362:bool[])
            n163 = And Array Elements(Boolean array=w357) -> (logical AND=w354:bool)
            n164 = And Array Elements(Boolean array=w362) -> (logical AND=w361:bool)
            n165 = Bundle By Name(cluster=w365, "SearchOnlyTopVIs"=w354, "SearchOnlyClasses"=w361, "SearchDirs"=w358) -> (w364:T10)
            n166 = call <resource>:"UMLEditor ControlBusyDialog.vi"("Title/StatusText"="Starts loading VIs", "error in (no error)"=w353) -> ("error out"=w351:errorcluster)  [unwired: 2 in, 15 out]
            n167 = stacked-sequence {
              tunnel: [w368] -> w350
              tunnel: w351 -> [w368]
              frame #0 {
                n168 = Wait (ms)(milliseconds to wait=u32 50) -> ()  [unwired: 1 out]
              }
            }
          }
          frame "GetClassRelationShips" {
            w404 = enum16{"Update", "ReadFromFile", "SaveToFile"}."SaveToFile" ("Actions")
            (unwired) inf
            n169 = Unbundle By Name(w420) -> ("SearchOnlyTopVIs"=w412:bool, "SearchOnlyClasses"=w413:bool, "SearchDirs"=w411:path[], "dependencyClassPath"=w418:path[])
            n170 = while {
              shift-right: [w440] -> w405
              shift-left: w419 -> [w441]
              shift-right: [w439] -> _
              shift-left: w418 -> [w445]
              shift-right: [w453] -> w417
              shift-left: w409 -> [w454]
              tunnel: w416 -> [w446]
              shift-right: [w451] -> w415
              shift-left: w410 -> [w452]
              tunnel: w411 -> [w449]
              tunnel: w413 -> [w448]
              tunnel: w414 -> [w443]
              tunnel: w412 -> [w442]
              shift-right: [w435] -> _
              shift-left: path[] [] -> [w435]
              tunnel: w407 -> [w429]
              tunnel: w406 -> [w428]
              tunnel: w403 -> [w423]
              i -> [w426]
              stop <- w431 stop-if-true
              # "Use later to keep track of what class that has been synced"
              n171 = call <resource>:"ReversedEngineering FilterClassSearch.vi"("dependencyClassPath"=w445, "LoopIteration"=w426, "IgnoreClasses"=w429, "error in (no error)"=w441, "SerachDirs"=w449, "Only Create this/these classes and its dependencis"=w446, "SearchOnlyClasses"=w448, "Only analyse this class methods and attributes(False)"=w443, "SearchOnlyTopVIs"=w442, "SyncOption"=w428) -> ("dependencyClassPathOut"=w444:path[], "AnalyseClass"=w447:bool, "AnalyseDone"=w430:bool, "ClassPathToAnalyse"=w434:path, "error out"=w437:errorcluster)  [unwired: 1 in, 4 out]
              n172 = call <vilib>:"Get File Extension.vi"("file"=w434) -> ("filename without extension"=w433:string)  [unwired: 1 in, 9 out]
              n173 = Increment(x=w426) -> (x+1=w425:i32)
              n174 = case shown="True" w447 {
                tunnel: w437 -> [w478 w486]
                tunnel: w454 -> [w479 w498]
                tunnel: [w479 w497] -> w453
                tunnel: w443 -> [_ w495]
                tunnel: w452 -> [w480 w494]
                tunnel: [w480 w493] -> w451
                tunnel: [_ w490] -> w450
                tunnel: w434 -> [_ w489]
                tunnel: [w478 w487] -> w436
                tunnel: w433 -> [_ w485]
                tunnel: [_ w484] -> w432
                tunnel: w423 -> [_ w481]
                frame False {
                }
                frame True {
                  n175 = Strip Path(path=w489) -> (name=w482:string)  [unwired: 1 out]
                  n176 = call <resource>:"ReversedEngineering GetClassDependencyInfo.vi"("Class/Create Path"=w489, "error in (no error)"=w486, "AttributeSerachP{atternNamesToIgnore"=w481, "Only analyse this class methods and attributes(False)"=w495) -> ("classInfo"=w490:T7, "TypeDefs"=w496:T3[], "error out"=w483:errorcluster)  [unwired: 13 out]
                  n177 = Unbundle By Name(w483) -> ("code"=w488:i32)
                  n178 = case shown="Error" w483 {
                    selector: w483 -> [_ w499]
                    tunnel: w482 -> [_ w500]
                    frame No Error {
                    }
                    frame Error {
                      n179 = call <resource>:"GOOP_DebugLogger.vi"("error in (no error)"=w499, "State"=w500) -> ()  [unwired: 7 in, 3 out]
                    }
                  }
                  n180 = Match Pattern(string=w482, regular expression="[.][cC][tT][lLtT]$") -> (offset past match=w491:i32)  [unwired: 4 out]
                  n181 = case shown="6100" w488 {
                    tunnel: w489 -> [_ _ w510 _]
                    tunnel: w483 -> [w505 w506 _ w514]
                    tunnel: [w505 w506 w508 w514] -> w487
                    tunnel: w486 -> [_ _ w508 _]
                    tunnel: w485 -> [_ _ _ w513]
                    tunnel: [_ _ _ w512] -> w484
                    frame 6100 {
                    }
                    frame Default {
                    }
                    frame 1..6099, 6101..6999, 7001.. {
                      n182 = Format Into String(format string="WARNING\nClass: %s\nCould not be completely analysed.\nThis class might have been removed from the current project.", w510) -> (resulting string=w509:string)  [unwired: 2 in, 1 out]
                      n183 = One Button Dialog(message=w509) -> ()  [unwired: 2 out]
                    }
                    frame 7000 {
                      n184 = Format Into String(format string="This class: %s could not be found in the current project.", w513) -> (resulting string=w516:string)  [unwired: 2 in, 1 out]
                      n185 = One Button Dialog(message=w516, button name ("OK")="Abort") -> (true=w512:bool)
                    }
                  }
                  n186 = case shown="-1" w491 {
                    tunnel: w490 -> [_ w504]
                    tunnel: w494 -> [w501 w503]
                    tunnel: [w501 w502] -> w493
                    frame 0, Default {
                    }
                    frame -1 {
                      n187 = Build Array (concatenate)(w503, w504) -> (w502:T7[])
                    }
                  }
                  n188 = Build Array (concatenate)(w498, w496) -> (w497:T3[])
                }
              }
              n189 = call <resource>:"UMLEditor ControlBusyDialog.vi"("I-Value"=w425, "Action(SendStatusMessage)"=UMLEditor_BusyDialogAction."Send_I-Value") -> ()  [unwired: 2 in, 16 out]
              n190 = Unbundle By Name(w450) -> ("baseClasses"=w458:path[], "compAggClasses"=w457:path[], "aggClasses"=w456:path[], "depClasses"=w455:path[], "ParentInterfaces"=w424:path[])
              n191 = Or(x=w432, y=w430) -> (x .or. y?=w431:bool)
              n192 = Build Array (concatenate)(w444, w458, w457, w456, w455, w424) -> (w459:path[])
              n193 = for {
                shift-right: [w521] -> w439
                shift-left: path[] [] -> [w522]
                tunnel: w459 -> [w519] mode=indexing
                n194 = Search 1D Array(1D array=w522, element=w519) -> (index of element=w520:i32)  [unwired: 1 out]
                n195 = Empty String/Path?(string/path=w519) -> (empty?=w517:bool)
                n196 = Greater Or Equal To 0?(x=w520) -> (x >= 0?=w523:bool)
                n197 = Or(x=w523, y=w517) -> (x .or. y?=w518:bool)
                n198 = case shown="False" w518 {
                  tunnel: w519 -> [w526 _]
                  tunnel: w522 -> [w525 w527]
                  tunnel: [w524 w527] -> w521
                  frame False {
                    n199 = Build Array (concatenate)(w525, w526) -> (w524:path[])
                  }
                  frame True {
                  }
                }
              }
              n200 = Array Size(array=w439) -> (size(s)=w438:i32)
              n201 = case shown="False" w430 {
                tunnel: [w463 w472] -> w440
                tunnel: w426 -> [w461 w471]
                tunnel: w438 -> [_ w470]
                tunnel: w436 -> [w462 w469]
                frame True {
                  n202 = Format Into String(format string="Analysing Class/Type: %d of %d", w461, w461) -> (resulting string=w466:string)  [unwired: 2 in, 1 out]
                  n203 = call <resource>:"UMLEditor ControlBusyDialog.vi"("Title/StatusText"=w466, "error in (no error)"=w462) -> ("error out"=w464:errorcluster)  [unwired: 2 in, 15 out]
                  n204 = call <resource>:"UMLEditor ControlBusyDialog.vi"("error in (no error)"=w464, "Action(SendStatusMessage)"=UMLEditor_BusyDialogAction."GetBusyDialogStatus") -> ("error out"=w463:errorcluster)  [unwired: 2 in, 15 out]
                }
                frame False {
                  n205 = Increment(x=w471) -> (x+1=w476:i32)
                  n206 = Wait (ms)(milliseconds to wait=u32 5) -> ()  [unwired: 1 out]
                  n207 = Format Into String(format string="Analysing Class/Type: %d of %d", w476, w470) -> (resulting string=w475:string)  [unwired: 2 in, 1 out]
                  n208 = call <resource>:"UMLEditor ControlBusyDialog.vi"("Title/StatusText"=w475, "error in (no error)"=w469) -> ("error out"=w473:errorcluster)  [unwired: 2 in, 15 out]
                  n209 = call <resource>:"UMLEditor ControlBusyDialog.vi"("error in (no error)"=w473, "Action(SendStatusMessage)"=UMLEditor_BusyDialogAction."GetBusyDialogStatus") -> ("error out"=w472:errorcluster)  [unwired: 2 in, 15 out]
                }
              }
            }
            n210 = Bundle By Name(cluster=w420, "classInfos"=w415, "TypeDefs"=w417) -> (w421:T10)
            n211 = call <resource>:"GOOP_AnalyseMethodCache.vi"("Actions"=w404, "error in (no error)"=w405) -> ()  [unwired: 7 in, 3 out]
            n212 = call <resource>:"GOOP_AnalyseAttributeCache.vi"("Actions"=w404, "error in (no error)"=w405) -> ()  [unwired: 7 in, 3 out]
          }
          frame "RemoveDublicateTypes" {
            n213 = Unbundle By Name(w531) -> ("TypeDefs"=w533:T3[])
            n214 = for {
              tunnel: w533 -> [w548] mode=indexing
              shift-right: [w547] -> _
              shift-left: path[] [] -> [w546]
              shift-right: [w543] -> w534
              shift-left: i32[] [] -> [w542]
              i -> [w541]
              n215 = Unbundle By Name(w548) -> ("TypeDefPath"=w545:path)
              n216 = Search 1D Array(1D array=w546, element=w545) -> (index of element=w544:i32)  [unwired: 1 out]
              n217 = case shown="-1" w544 {
                tunnel: [w551 w552] -> w543
                tunnel: w542 -> [w550 w552]
                tunnel: w541 -> [w549 _]
                frame 0, Default {
                  n218 = Build Array (concatenate)(w550, w549) -> (w551:i32[])
                }
                frame -1 {
                }
              }
              n219 = Build Array (concatenate)(w546, w545) -> (w547:path[])
            }
            n220 = Reverse 1D Array(array=w534) -> (reversed array=w532:i32[])
            n221 = for {
              shift-right: [w539] -> w530
              shift-left: w533 -> [w540]
              tunnel: w532 -> [w538] mode=indexing
              n222 = Delete From Array(array=w540, index=w538) -> (array with subset deleted=w539:T3[])  [unwired: 1 in, 1 out]
            }
            n223 = Bundle By Name(cluster=w531, "TypeDefs"=w530) -> (w529:T10)
          }
          frame "RemoveClassDependenciesDueToInheritance" {
            n224 = Unbundle By Name(w561) -> ("classInfos"=w558:T7[])
            n225 = for {
              tunnel: w558 -> [w569] mode=indexing
              tunnel: w558 -> [w584] mode=indexing
              tunnel: w558 -> [w582]
              tunnel: w558 -> [w571]
              tunnel: [w574] -> w557 mode=indexing
              n226 = Unbundle By Name(w584) -> ("baseClasses"=w564:path[], "ParentInterfaces"=w563:path[])
              n227 = Unbundle By Name(w569) -> ("noOfAgg"=w568:i32[])
              n228 = Unbundle By Name(w569) -> ("depClasses"=w579:path[], "aggClasses"=w580:path[], "compAggClasses"=w583:path[])
              n229 = for {
                tunnel: w583 -> [w619] mode=indexing
                tunnel: w582 -> [w618]
                shift-right: [w616] -> w578
                shift-left: path[] [] -> [w615]
                n230 = call <resource>:"ReversedEngineering GetInheritanceClasses.vi"("classInfos"=w618, "classPath"=w619) -> ("baseClasses"=w617:path[])  [unwired: 17 out]
                n231 = Build Array (concatenate)(w617, w615) -> (w616:path[])
              }
              n232 = Build Array (concatenate)(w564, w563) -> (w562:path[])
              n233 = call <resource>:"ReversedEngineering RemoveThesePathes.vi"("classesIn"=w580, "removeThese"=w578) -> ("classesOut"=w572:path[], "Removed(Index-1*n)"=w570:i32[])  [unwired: 16 out]
              n234 = for {
                tunnel: w570 -> [w588] mode=indexing
                shift-right: [w586] -> w567
                shift-left: w568 -> [w585]
                n235 = Delete From Array(array=w585, length=1, index=w588) -> (array with subset deleted=w586:i32[])  [unwired: 1 out]
              }
              n236 = for {
                tunnel: w572 -> [w594] mode=indexing
                tunnel: w572 -> [w602]
                shift-right: [w597] -> w575
                shift-left: path[] [] -> [w598]
                tunnel: w571 -> [w593]
                shift-right: [w589] -> w565
                shift-left: i32[] [] -> [w591]
                tunnel: w567 -> [w590] mode=indexing
                i -> [w601]
                n237 = call <resource>:"ReversedEngineering GetInheritanceClasses.vi"("classInfos"=w593, "classPath"=w594) -> ("baseClasses"=w592:path[])  [unwired: 17 out]
                n238 = Delete From Array(array=w602, length=1, index=w601) -> (array with subset deleted=w599:path[])  [unwired: 1 out]
                n239 = for {
                  tunnel: w599 -> [w612]
                  tunnel: w592 -> [w613] mode=indexing
                  tunnel: [w611] -> w596 mode=indexing
                  n240 = Search 1D Array(1D array=w612, element=w613) -> (index of element=w614:i32)  [unwired: 1 out]
                  n241 = Greater Or Equal To 0?(x=w614) -> (x >= 0?=w611:bool)
                }
                n242 = Or Array Elements(Boolean array=w596) -> (logical OR=w595:bool)
                n243 = case shown="False" w595 {
                  tunnel: w598 -> [w608 w610]
                  tunnel: [w607 w610] -> w597
                  tunnel: w594 -> [w606 _]
                  tunnel: w591 -> [w605 w609]
                  tunnel: w590 -> [w604 _]
                  tunnel: [w603 w609] -> w589
                  frame False {
                    n244 = Build Array (concatenate)(w605, w604) -> (w603:i32[])
                    n245 = Build Array (concatenate)(w608, w606) -> (w607:path[])
                  }
                  frame True {
                  }
                }
              }
              n246 = call <resource>:"ReversedEngineering RemoveThesePathes.vi"("classesIn"=w579, "removeThese"=w578) -> ("classesOut"=w577:path[])  [unwired: 17 out]
              n247 = call <resource>:"ReversedEngineering RemoveThesePathes.vi"("classesIn"=w577, "removeThese"=w562) -> ("classesOut"=w573:path[])  [unwired: 17 out]
              n248 = Bundle By Name(cluster=w569, "depClasses"=w573, "aggClasses"=w575, "noOfAgg"=w565) -> (w574:T7)
            }
            n249 = Bundle By Name(cluster=w561, "classInfos"=w557) -> (w560:T10)
            n250 = Select(t="AddApplicationNodes" ("y"), s=w553, f="Exit" ("y")) -> (s? t:f=w555:string)
          }
          frame "AddApplicationNodes" {
            n251 = Unbundle By Name(w630) -> ("classInfos"=w627:T7[], "dependencyClassPath"=w625:path[], "TopVIPath"=w624:path)
            n252 = Empty String/Path?(string/path=w624) -> (empty?=w623:bool)
            n253 = Bundle By Name(cluster=T7 {"classPath"=path "", "inherits"=FALSE, "baseClasses"=[], "compAggClasses"=[], "noOfCompObj"=[], "aggClasses"=[], "noOfAgg"=[], "depClasses"=[], "methods"=[], "methodPuplic"=[], "objectAttrib"=[], "classAttrib"=[], "ClassDesc"="", "DependencyDetails"=[], "Interface"=FALSE, "ParentInterfaces"=[]} ("classInfo"), "ClassDesc"="<<APPLICATION>>") -> (w621:T7)
            n254 = case shown="False" w623 {
              tunnel: w627 -> [w637 w638]
              tunnel: [w636 w638] -> w626
              tunnel: w621 -> [w635 _]
              tunnel: w625 -> [w634 _]
              tunnel: w624 -> [w632 _]
              frame False {
                n255 = Bundle By Name(cluster=w635, "depClasses"=w634, "classPath"=w632) -> (w633:T7)
                n256 = Build Array (concatenate)(w633, w637) -> (w636:T7[])
              }
              frame True {
              }
            }
            n257 = Bundle By Name(cluster=w630, "classInfos"=w626) -> (w629:T10)
          }
          frame "Error", Default {
          }
        }
        n258 = Unbundle By Name(w69) -> ("status"=w65:bool)
        n259 = Equal?(x=w68, y="Exit") -> (x = y?=w66:bool)
        n260 = Or(x=w66, y=w65) -> (x .or. y?=w64:bool)
      }
    }
    frame Error {
    }
  }
  n261 = Unbundle By Name(w26) -> ("TypeDefs"=w14:T3[], "classInfos"=w13:T7[], "VIRef"=w22:refnum<vi>[])
  n262 = call <resource>:"Error_ClearError.vi"("codes"=i32[] [6100, 7000], "error in (no error)"=w17) -> ("Cleared?"=w15:bool, "error out"=→"error out":errorcluster)  [unwired: 3 in, 13 out]
  "Cancelled" <- w15
  n263 = call <resource>:"Common_ ViCacheMemory.vi"("ViRef-Array"=w22) -> ()  [unwired: 3 in, 16 out]
  n264 = case shown="True" w15 {
    tunnel: w14 -> [w644 _]
    tunnel: w13 -> [w643 _]
    tunnel: [w644 _] -> w12
    tunnel: [w643 _] -> w11
    frame False {
    }
    frame True {
    }
  }
  "classInfos" <- w11
  "TypeDefs" <- w12
